vi "Control Cluster(SubVI).vi"(10 "Control cluster In New":T1, 11 "Control cluster In Original":T1) -> (3 "Control cluster Out":T1)   [LabVIEW 2014]
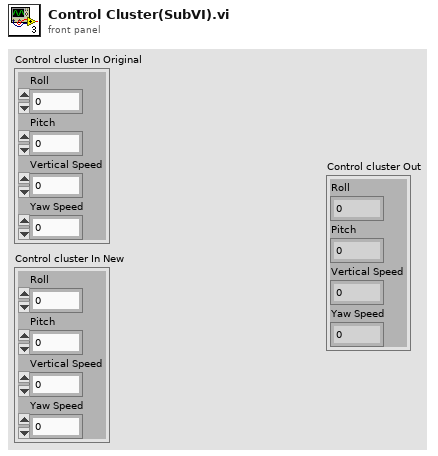
[diagram p1: front panel]
types:
  T1 = cluster{"Roll":dbl, "Pitch":dbl, "Vertical Speed":dbl, "Yaw Speed":dbl}
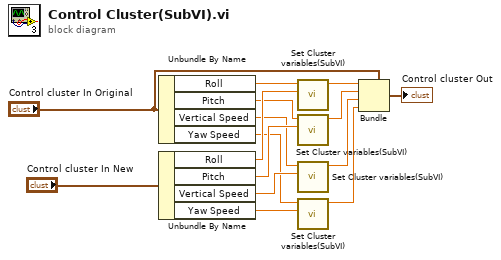
[diagram p0: block diagram]
diagram:
  n1 = Unbundle By Name("Control cluster In Original") -> ("Roll"=w13:dbl, "Pitch"=w11:dbl, "Vertical Speed"=w9:dbl, "Yaw Speed"=w6:dbl)
  n2 = Unbundle By Name("Control cluster In New") -> ("Roll"=w14:dbl, "Pitch"=w10:dbl, "Vertical Speed"=w8:dbl, "Yaw Speed"=w7:dbl)
  n3 = call "Set Cluster variables(SubVI).vi"("In new"=w14, "In original"=w13) -> ("Out"=w2:dbl)  [unwired: 9 in]
  n4 = call "Set Cluster variables(SubVI).vi"("In new"=w10, "In original"=w11) -> ("Out"=w1:dbl)  [unwired: 9 in]
  n5 = call "Set Cluster variables(SubVI).vi"("In new"=w8, "In original"=w9) -> ("Out"=w5:dbl)  [unwired: 9 in]
  n6 = call "Set Cluster variables(SubVI).vi"("In new"=w7, "In original"=w6) -> ("Out"=w4:dbl)  [unwired: 9 in]
  n7 = Bundle(cluster="Control cluster In Original", "Roll"=w2, "Pitch"=w1, "Vertical Speed"=w5, "Yaw Speed"=w4) -> (→"Control cluster Out":T1)
